vi "Get Minimum Trigger Interval.vi"(8 "error in (no error)":errorcluster, 11 "HamamatsuFluor in":refnum<class "HamamatsuFluor.lvclass">) -> (0 "error out":errorcluster, 2 "Minimum Interval (ms)":dbl, 3 "HamamatsuFluor out":refnum<class "HamamatsuFluor.lvclass">)   [LabVIEW 2020, in "DAQ Timed SPIM.lvlib" / "HamamatsuFluor_v2.lvlib" / "HamamatsuFluor.lvclass"]
uses:
  HamamatsuFluor.lvclass
  HamamatsuFluor.lvclass/HamamatsuFluor.ctl
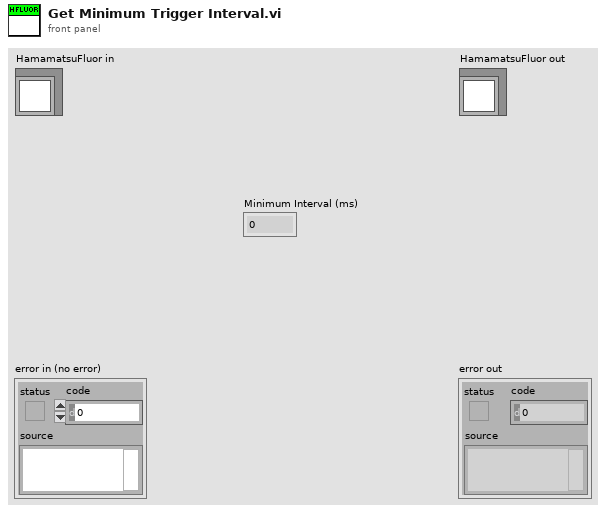
[diagram p1: front panel]
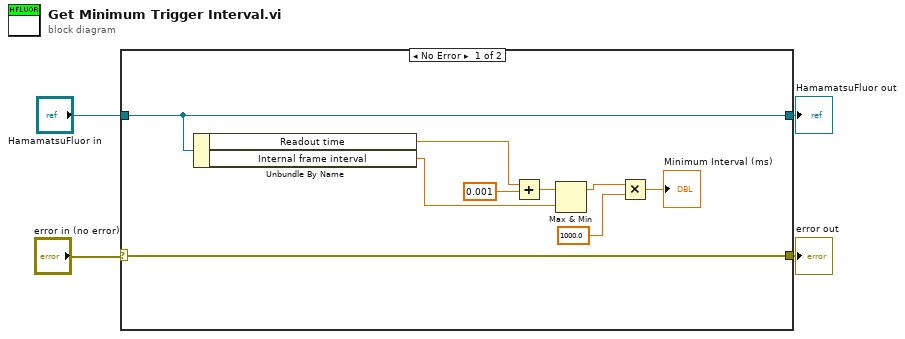
[diagram p0: block diagram]
diagram:
  n1 = case shown="No Error" "error in (no error)" {
    selector: "error in (no error)" -> [w11 w14]
    tunnel: "HamamatsuFluor in" -> [w10 w15]
    tunnel: [w11 w14] -> w2
    tunnel: [w10 w15] -> w1
    frame No Error {
      n2 = Unbundle By Name(w10) -> ("Readout time"=w6:dbl, "Internal frame interval"=w7:dbl)
      n3 = Add(x=w6, y=0.001 ("x")) -> (x+y=w12:dbl)
      n4 = Max & Min(x=w12, y=w7) -> (max(x,y)=w5:dbl)  [unwired: 1 out]
      n5 = Multiply(x=w5, y=1000.0) -> (x*y=→"Minimum Interval (ms)":dbl)
    }
    frame Error {
    }
  }
  "error out" <- w2
  "HamamatsuFluor out" <- w1
